vi "PLC_Open.vi"(2 "COM Port":refnum<visa-resource-name>, 8 "error in (no error)":errorcluster, 9 "Port":u16, 10 "Host":string, 11 "Transport":enum16{"TCP", "COM"}(ring)) -> (0 "error out":errorcluster, 3 "PLC Conn":refnum<visa-resource-name>)   [LabVIEW 2018]
doc: "Use this template to build a VI to use as a subVI."
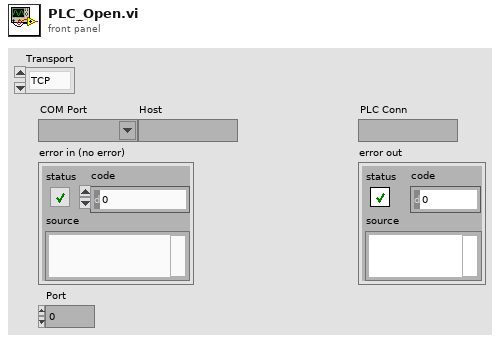
[diagram p1: front panel]
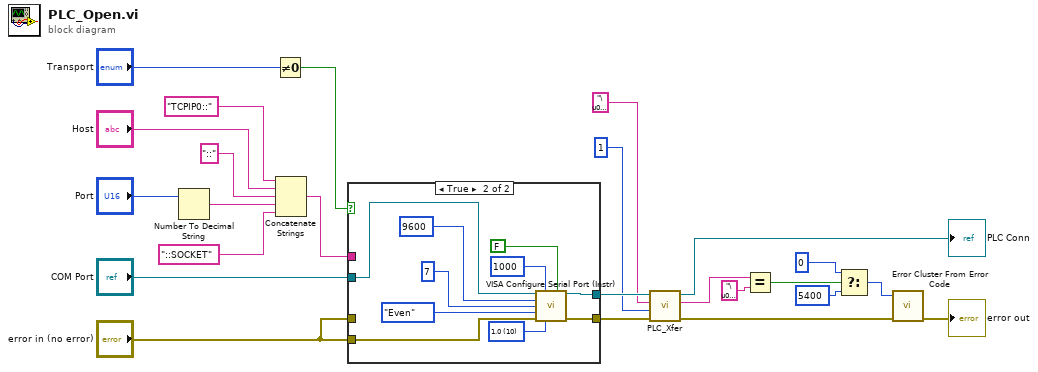
[diagram p0: block diagram]
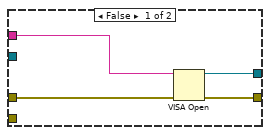
[diagram p2: hidden frame]
diagram:
  n1 = Number To Decimal String(number="Port") -> (decimal integer string=w19:string)  [unwired: 1 in]
  n2 = Not Equal To 0?(x="Transport") -> (x != 0?=w17:bool)
  n3 = Concatenate Strings("TCPIP0::", "Host", "::", w19, "::SOCKET") -> (w16:string)
  n4 = case shown="True" w17 {
    tunnel: w16 -> [w28 _]
    tunnel: "error in (no error)" -> [w27 _]
    tunnel: "COM Port" -> [_ w38]
    tunnel: "error in (no error)" -> [_ w37]
    tunnel: [w26 w30] -> w13
    tunnel: [w25 w29] -> w12
    frame False {
      n5 = VISA Open(error in (no error)=w27, VISA resource name=w28) -> (VISA resource name=w26:refnum<visa-resource-name>, error out=w25:errorcluster)  [unwired: 3 in]
    }
    frame True {
      w33 = u16 10 items=["1.0"=10, "1.5"=15, "2.0"=20] ("stop bits (10: 1 bit)")
      n6 = call <vilib>:"VISA Configure Serial Port (Instr).vi"("VISA resource name"=w38, "timeout (10sec)"=u32 1000, "Enable Termination\nChar (T)"=FALSE, "baud rate (9600)"=u32 9600, "data bits (8)"=u16 7, "parity (0:none)"=enum16{"None", "Odd", "Even", "Mark", "Space"}."Even", "error in (no error)"=w37, "stop bits (10: 1 bit)"=w33) -> ("VISA resource name out"=w30:refnum<visa-resource-name>, "error out"=w29:errorcluster)  [unwired: 6 in]
    }
  }
  n7 = call "PLC_Xfer.vi"("error in (no error)"=w12, "RX Bytes"=u32 1, "TX"="\u0005", "PLC Conn"=w13) -> ("error out"=w3:errorcluster, "RX"=w9:string, "PLC Conn out"=→"PLC Conn":refnum<visa-resource-name>)  [unwired: 5 in]
  n8 = Equal?(x=w9, y="\u0006") -> (x = y?=w7:bool)
  n9 = Select(t=0, s=w7, f=5400) -> (s? t:f=w4:i32)
  n10 = call <vilib>:"Error Cluster From Error Code.vi"("error in (no error)"=w3, "error code (0)"=w4) -> ("error out"=→"error out":errorcluster)  [unwired: 7 in]
